vi "Add Default Arguments On Error.vi"(4 "Target_Type? (T)":bool=TRUE, 5 "Caller (This VI.Name)":string, 6 "timestamp? (T)":bool=TRUE, 7 "convert to warning? (F)":bool, 9 "error in (no error)":errorcluster, 11 "error arguments (\"\")":string) -> (1 "error out":errorcluster)   [LabVIEW 2019, in "Error Generation.lvlib"]
doc: "If \"error in\" is an error, then add arguments:\n\n<b>timestamp?</b>\nadd a current date & time string to the error description.\n<b>convert to warning?</b>\nconvert the error into a warning (error.status=false)\n<b>error arguments</b>\nInsert an argument name and data in this format: argument=argument data\nMultiple Arguments can be inserted EOL separated.\nUse arguments, to specify the error more detailled.\n- - -\nCopyright (c) 2023, Merecs Engineering GmbH"
uses:
  Error Generation.lvlib
  support/Convert Argument Representation.vi
  Add Argument.vi
panel:
  # "Connector Pane"
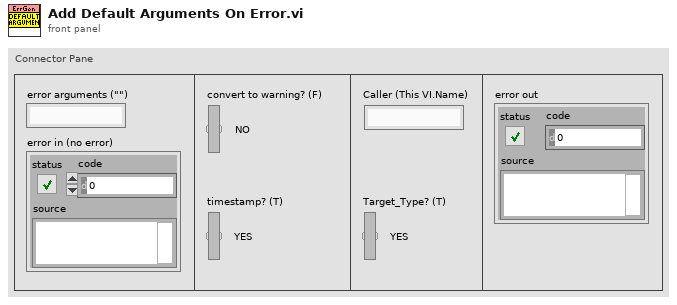
[diagram p1: front panel]
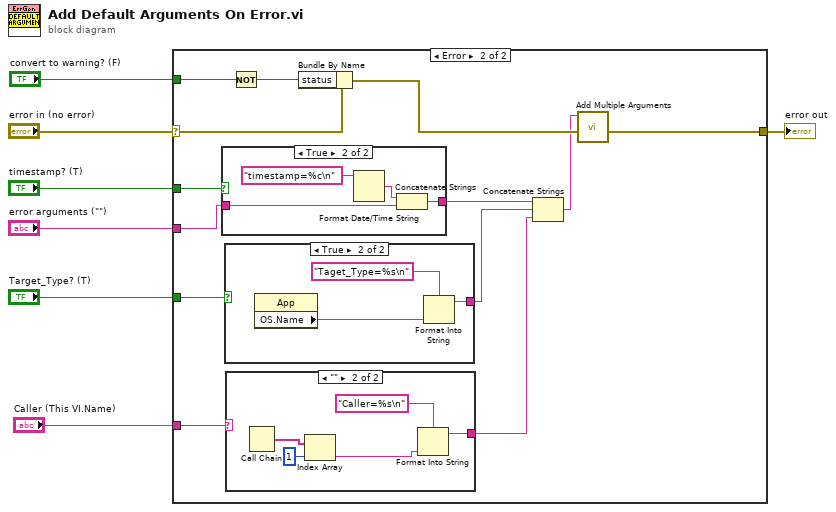
[diagram p0: block diagram]
diagram:
  n1 = case shown="Error" "error in (no error)" {
    selector: "error in (no error)" -> [w8 w21]
    tunnel: "timestamp? (T)" -> [_ w20]
    tunnel: "error arguments (\"\")" -> [_ w19]
    tunnel: [w8 w15] -> w4
    tunnel: "convert to warning? (F)" -> [_ w18]
    tunnel: "Target_Type? (T)" -> [_ w12]
    tunnel: "Caller (This VI.Name)" -> [_ w10]
    frame No Error {
    }
    frame Error {
      n2 = case shown="True" w20 {
        tunnel: w19 -> [w30 w32]
        tunnel: [w30 w31] -> w14
        frame False {
        }
        frame True {
          n3 = Format Date/Time String(time format string (%c)="timestamp=%c\n") -> (date/time string=w33:string)  [unwired: 2 in]
          n4 = Concatenate Strings(w33, w32) -> (w31:string)
        }
      }
      n5 = case shown="True" w12 {
        tunnel: [_ w28] -> w11
        frame False {
        }
        frame True {
          n6 = property class="App"() -> ("OS.Name"=w27:string)  [unwired: 2 in, 2 out]
          n7 = Format Into String(format string="Taget_Type=%s\n" ("time format string (%c)"), w27) -> (resulting string=w28:string)  [unwired: 2 in, 1 out]
        }
      }
      n8 = case shown="\"\"" w10 {
        tunnel: [_ w23] -> w9
        frame "False", Default {
        }
        frame "" {
          n9 = Call Chain() -> (call chain=w26:string[])
          n10 = Index Array(array=w26, index=1) -> (element=w24:string)
          n11 = Format Into String(format string="Caller=%s\n" ("time format string (%c)"), w24) -> (resulting string=w23:string)  [unwired: 2 in, 1 out]
        }
      }
      n12 = Not(x=w18) -> (.not. x?=w17:bool)
      n13 = Bundle By Name(cluster=w21, "status"=w17) -> (w16:errorcluster)
      n14 = Concatenate Strings(w14, w11, w9) -> (w13:string)
      n15 = call "Add Multiple Arguments.vi"("error in (no error)"=w16, "error arguments"=w13) -> ("error out"=w15:errorcluster)  [unwired: 9 in]
    }
  }
  "error out" <- w4
